vi "Obtain Topic.vi"(8 "error in (no error)":errorcluster, 9 "Region":T1, 10 "Name":string, 11 "AWS Credentials":T2) -> (0 "error out":errorcluster, 3 "Topic out":refnum<class "Topic.lvclass">)   [LabVIEW 2015, in "NI_AWS_SNS.lvlib" / "Topic.lvclass"]
doc: "Returns the requested topic object."
uses:
  Topic.lvclass
  Core/HTTP Request/AWS Credentials.ctl
  Core/HTTP Request/Region.ctl
  Core/HTTP Request/HTTP Request.lvclass
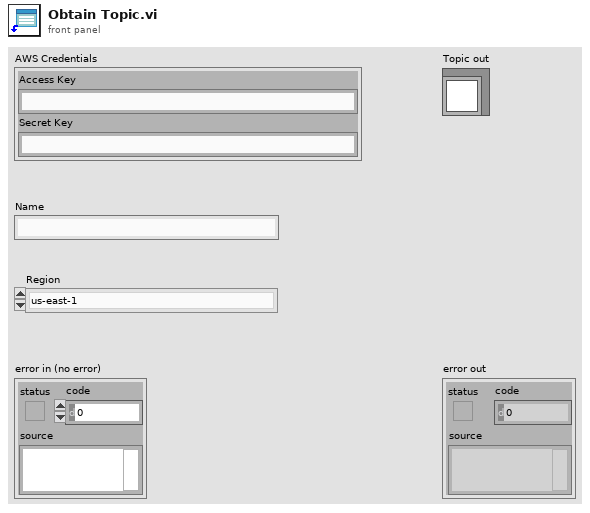
[diagram p1: front panel]
types:
  T1 = typedef "NI_AWS_Core.lvlib/HTTP Request.lvclass/Region.ctl" = enum16{"us-east-1", "us-east-2", "us-west-1", "us-west-2", "ap-northeast-1", "ap-northeast-2", "ap-southeast-1", "ap-southeast-2", "ca-central-1", "eu-central-1", "eu-west-1", "eu-west-2", "sa-east-1"}
  T2 = typedef "NI_AWS_Core.lvlib/HTTP Request.lvclass/AWS Credentials.ctl" = cluster{"Access Key":string, "Secret Key":string}
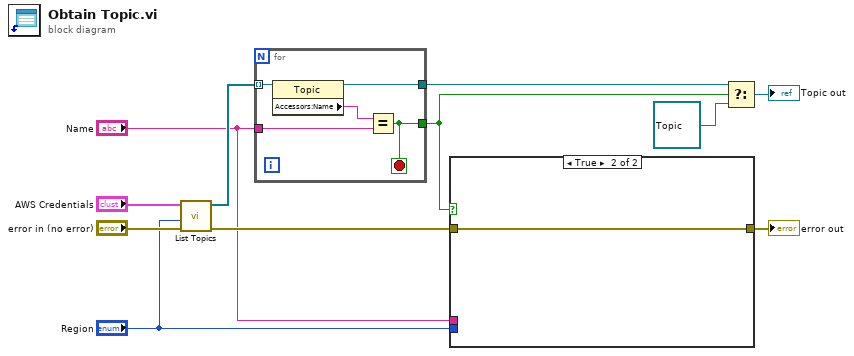
[diagram p0: block diagram]
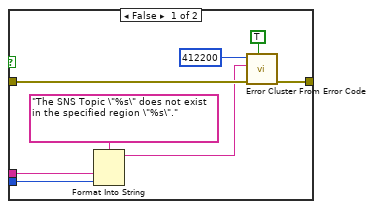
[diagram p2: hidden frame]
diagram:
  n1 = call "List Topics.vi"("error in (no error)"="error in (no error)", "Region"="Region", "AWS Credentials"="AWS Credentials") -> ("error out"=w6:errorcluster, "Topics out"=w9:refnum<class "Topic.lvclass">[])  [unwired: 7 in]
  n2 = for {
    tunnel: w9 -> [w16] mode=indexing
    tunnel: "Name" -> [w14]
    tunnel: [w13] -> w3
    tunnel: [w12] -> w8
    stop <- w13 stop-if-true
    n3 = property class="Topic"(reference=w16) -> (reference out=w12:refnum<class "Topic.lvclass">, "Accessors:Name"=w15:string)  [unwired: 1 in, 1 out]
    n4 = Equal?(x=w15, y=w14) -> (x = y?=w13:bool)
  }
  n5 = case shown="True" w3 {
    tunnel: w6 -> [w23 w25]
    tunnel: [w24 w25] -> w5
    tunnel: "Name" -> [w19 _]
    tunnel: "Region" -> [w18 _]
    frame False {
      n6 = Format Into String(format string="The SNS Topic \"%s\" does not exist in the specified region \"%s\".", w19, w18) -> (resulting string=w17:string)  [unwired: 2 in, 1 out]
      n7 = call <vilib>:"Error Cluster From Error Code.vi"("show call chain? (False)"=TRUE, "error in (no error)"=w23, "error message (\"\")"=w17, "error code (0)"=412200) -> ("error out"=w24:errorcluster)  [unwired: 5 in]
    }
    frame True {
    }
  }
  "error out" <- w5
  n8 = Select(t=w8, s=w3, f=refnum<class "Topic.lvclass"> refnum ("SNS")) -> (s? t:f=→"Topic out":refnum<class "Topic.lvclass">)
